vi "getAll.vi"(6 "timeout (ms) [500]":i32=500, 8 "error in (no error)":errorcluster, 11 "Instrument in":refnum<class "Instrument.lvclass">) -> (0 "error out":errorcluster, 1 "getAll":variant, 3 "Instrument out":refnum<class "Instrument.lvclass">)   [LabVIEW 2019, in "Instrument.lvlib" / "Instrument.lvclass"]
doc: "Send \"getAll\" command to remote Instrument. Returns contents of \"getAll.ctl\""
uses:
  Instrument.lvclass
  Typedefs/Instrument.Commands--Enum.ctl
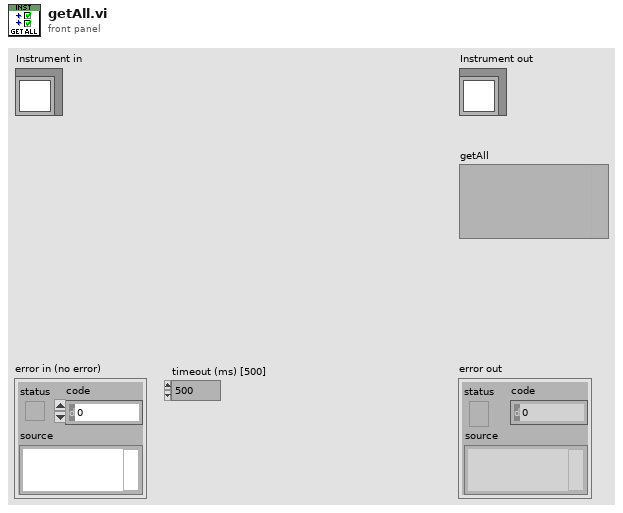
[diagram p1: front panel]
types:
  T1 = typedef "Instrument.lvlib/Instrument.lvclass/Instrument.Commands--Enum.ctl" = enum16{"ACK", "HELP", "IDN", "getAll", "getAllData"}
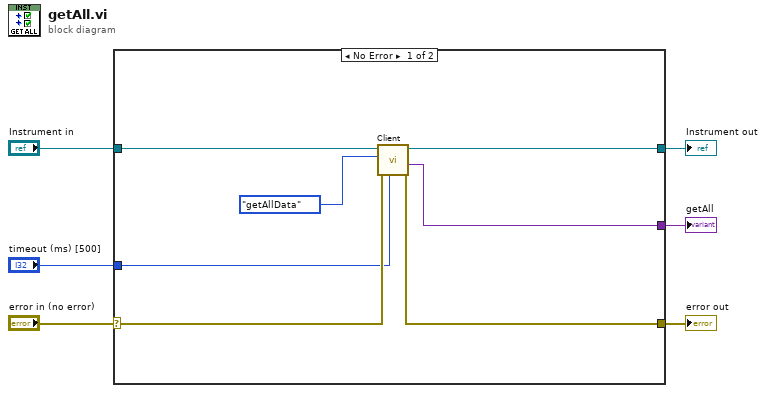
[diagram p0: block diagram]
diagram:
  n1 = case shown="No Error" "error in (no error)" {
    selector: "error in (no error)" -> [w11 w15]
    tunnel: [w8 w15] -> w5
    tunnel: [w10 w14] -> w3
    tunnel: "Instrument in" -> [w13 w14]
    tunnel: [w9 _] -> w2
    tunnel: "timeout (ms) [500]" -> [w7 _]
    frame No Error {
      n2 = call-dynamic "Client.vi"("timeout (ms) [500]"=w7, "error in (no error)"=w11, "Command in"=Instrument.Commands--Enum."getAllData" ("Commands"), "Instrument in"=w13) -> ("error out"=w8:errorcluster, "Data out"=w9:variant, "Instrument out"=w10:refnum<class "Instrument.lvclass">)  [unwired: 4 in, 1 out]
    }
    frame Error {
    }
  }
  "error out" <- w5
  "Instrument out" <- w3
  "getAll" <- w2
